vi "Analyze Code.vi"(11 "Test Case In":refnum<class "Runner Unit Test - Process Python Code.lvclass">) -> (0 "error out":errorcluster, 3 "Test Case Out":refnum<class "Runner Unit Test - Process Python Code.lvclass">)   [LabVIEW 2026, in "Runner Unit Test - Process Python Code.lvclass"]
uses:
  Runner Unit Test - Process Python Code.lvclass
  C:/Program Files/National Instruments/LabVIEW 2026/vi.lib/Astemes/LUnit/Test Case.lvclass
  Actors/Runner/Runner/Runner.lvclass
  Interfaces/IRunner/IRunner/Interfaces--cluster.ctl
  Interfaces/IProject Manager/IProject Manager.lvclass
  Interfaces/IFile Manager/IFile Manager.lvclass
  Interfaces/IPython Caller/IPython Caller.lvclass
  Interfaces/IElement Manager/IElement Manager.lvclass
  Interfaces/ILV File Creator/ILV File Creator.lvclass
  Interfaces/IHash Whitelist Handler/IHash Whitelist Handler.lvclass
  Actors/Mock Logger/Mock Logger/Mock Logger.lvclass
  C:/Program Files/National Instruments/LabVIEW 2026/vi.lib/ActorFramework/Actor/Actor.lvclass
  Type Definitions/Analysis Output--cluster.ctl
  Type Definitions/Type Definition--cluster.ctl
  Type Definitions/Parameter--cluster.ctl
  Type Definitions/Function--cluster.ctl
  <vilib>/ActorFramework/Message Enqueuer/Message Enqueuer.lvclass/Message Enqueuer.ctl
  <vilib>/ActorFramework/Message Enqueuer/Enqueue.vi
  Mocks/Mock IPython Caller/Mock IPython Caller.lvclass
  C:/Program Files/National Instruments/LabVIEW 2026/vi.lib/Astemes/LMock/Mock.lvclass
  C:/Users/juanj/Documents/hasbun_wood_engineering/github/py2vi/labview/Interfaces/IPython Caller/IPython Caller.lvclass
  <vilib>/ActorFramework/Stop Msg/Stop Msg.lvclass
  C:/Program Files/National Instruments/LabVIEW 2026/vi.lib/ActorFramework/Message/Message.lvclass
  <vilib>/Astemes/LMock/One Identical Inputs.vi
  <vilib>/ActorFramework/Message Priority Queue/Priority Enqueue.vi
  C:/Users/juanj/Documents/hasbun_wood_engineering/github/py2vi/labview/Mocks/Mock IPython Caller/Mock IPython Caller.lvclass
  Interfaces/IRunner/IRunner/IRunner.lvclass
  <vilib>/ActorFramework/Actor/Actor.lvclass
  <vilib>/Astemes/LMock/LMock Verifier.lvclass
  <vilib>/Astemes/LMock/LMock.lvlib
  <vilib>/Astemes/LMock/LMock One.lvlib
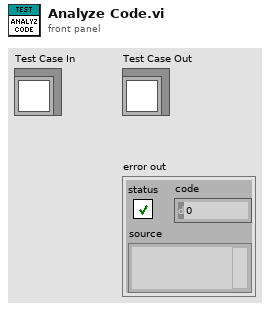
[diagram p1: front panel]
types:
  T1 = typedef "Function--cluster.ctl" = cluster{"name":string, "docstring":string, "input_parameters":T2[], "output_parameters":T2[]}
  T2 = typedef "Parameter--cluster.ctl" = cluster{"name":string, "data_type":string, "container":string, "dimensions":i32, "type_definition":string}
  T3 = typedef "Type Definition--cluster.ctl" = cluster{"name":string, "fields":T2[]}
  T4 = typedef "Analysis Output--cluster.ctl" = cluster{"type_definitions":T3[], "functions":T1[]}
  T5 = typedef "IRunner.lvlib/IRunner.lvclass/Interfaces--cluster.ctl" = cluster{"IProject Manager":refnum<class "IProject Manager.lvclass">, "IFile Manager":refnum<class "IFile Manager.lvclass">, "IPython Caller":refnum<class "IPython Caller.lvclass">, "IElement Manager":refnum<class "IElement Manager.lvclass">, "ILV File Creator":refnum<class "ILV File Creator.lvclass">, "IHash Whitelist Handler":refnum<class "IHash Whitelist Handler.lvclass">}
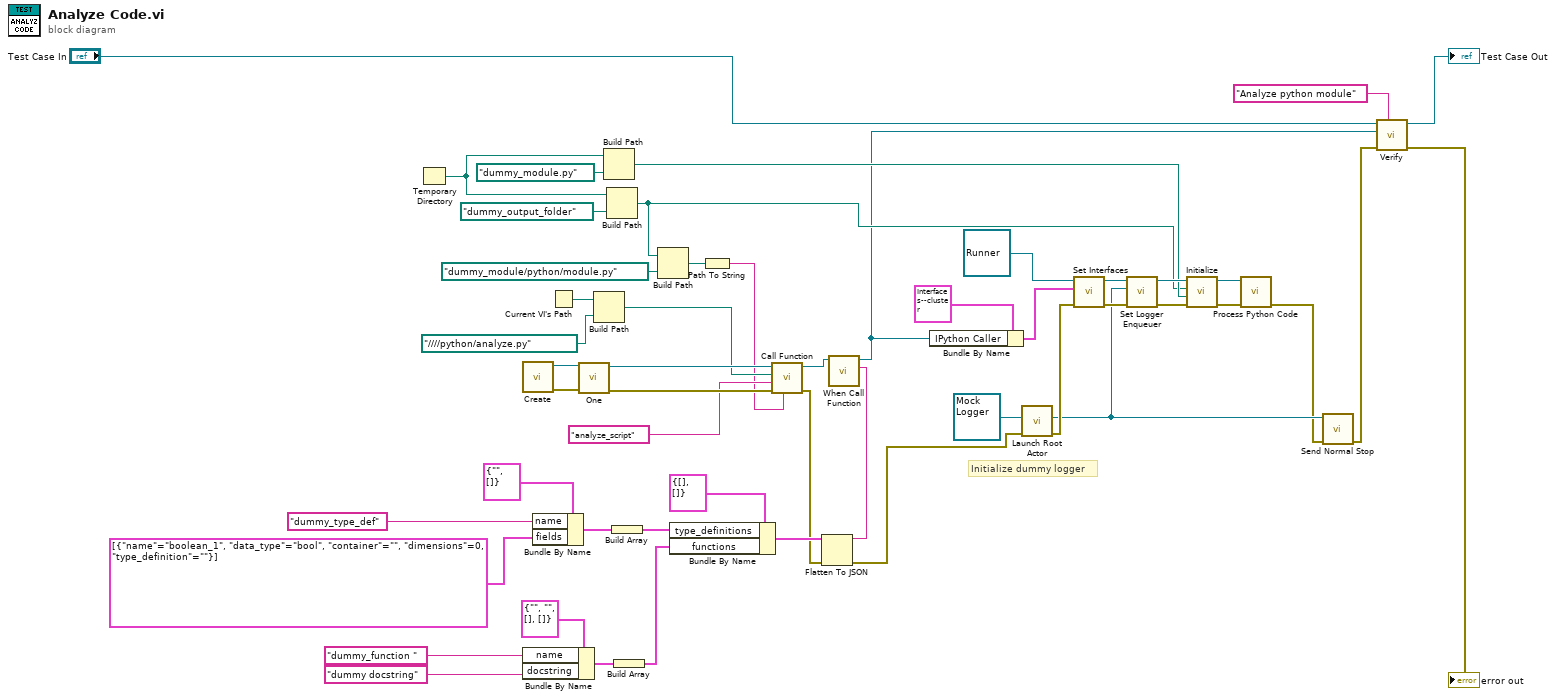
[diagram p0: block diagram]
diagram:
  # "Initialize dummy logger"
  n1 = Temporary Directory() -> (w36:path)
  n2 = call "Create.vi"() -> ("error out"=w30:errorcluster, "Mock Class Generator out"=w31:refnum<class "Mock IPython Caller.lvclass">)  [unwired: 10 in]
  n3 = Bundle By Name(cluster=T1 {"name"="", "docstring"="", "input_parameters"=[], "output_parameters"=[]} ("Function"), "name"="dummy_function ", "docstring"="dummy docstring") -> (w9:T1)
  n4 = Bundle By Name(cluster=T3 {"name"="", "fields"=[]} ("Type Definition"), "name"="dummy_type_def", "fields"=T2[] [{"name"="boolean_1", "data_type"="bool", "container"="", "dimensions"=0, "type_definition"=""}]) -> (w11:T3)
  n5 = Current VI's Path() -> (path=w26:path)
  n6 = call-poly <vilib>:"One.vi"("error in (no error)"=w30, "Mock in"=w31) -> ("error out"=w28:errorcluster, "Mock out"=w29:refnum<class "Mock IPython Caller.lvclass">)  [unwired: 8 in]
  n7 = Build Path(base path=w26, name or relative path=path "../../../../python/analyze.py") -> (appended path=w25:path)
  n8 = Build Path(base path=w36, name or relative path=path "dummy_module.py") -> (appended path=w37:path)
  n9 = Build Path(base path=w36, name or relative path=path "dummy_output_folder") -> (appended path=w23:path)
  n10 = Build Array(w11) -> (w10:T3[])
  n11 = Build Array(w9) -> (w8:T1[])
  n12 = Build Path(base path=w23, name or relative path=path "dummy_module/python/module.py") -> (appended path=w21:path)
  n13 = Bundle By Name(cluster=T4 {"type_definitions"=[], "functions"=[]} ("Analysis Output"), "type_definitions"=w10, "functions"=w8) -> (w7:T4)
  n14 = Path To String(path=w21) -> (string=w20:string)
  n15 = call-dynamic "Call Function.vi"("Input String"=w20, "error in"=w28, "Function"="analyze_script", "Python Script"=w25, "IPython Caller in"=w29) -> ("error out"=w4:errorcluster, "IPython Caller out"=w19:refnum<class "Mock IPython Caller.lvclass">)  [unwired: 4 in, 1 out]
  n16 = Flatten To JSON(anything=w7, error in (no error)=w4) -> (JSON string=w6:string, 11:w3:errorcluster)  [unwired: 1 in]
  n17 = call "When Call Function.vi"("Return String"=w6, "IPython Caller in"=w19) -> ("IPython Caller out"=w5:refnum<class "Mock IPython Caller.lvclass">)  [unwired: 9 in]
  n18 = Bundle By Name(cluster=T5 {"IProject Manager"=refnum, "IFile Manager"=refnum, "IPython Caller"=refnum, "IElement Manager"=refnum, "ILV File Creator"=refnum, "IHash Whitelist Handler"=refnum} ("Interfaces"), "IPython Caller"=w5) -> (w44:T5)
  n19 = call <vilib>:"Launch Root Actor.vi"("error in (no error)"=w3, "Actor"=refnum<class "Mock Logger.lvclass"> refnum ("Mock Logger.lvlib:Mock Logger.lvclass")) -> ("error out"=w50:errorcluster, "Actor's Enqueuer"=w42:refnum<class "Message Enqueuer.lvclass">)  [unwired: 8 in]
  n20 = call-dynamic "Set Interfaces.vi"("error in"=w50, "Interfaces"=w44, "Runner in"=refnum<class "Runner.lvclass"> refnum ("Runner.lvlib:Runner.lvclass")) -> ("error out"=w51:errorcluster, "Runner out"=w46:refnum<class "Runner.lvclass">)  [unwired: 7 in]
  n21 = call-dynamic "Set Logger Enqueuer.vi"("error in"=w51, "Logger"=w42, "Runner in"=w46) -> ("error out"=w48:errorcluster, "Runner out"=w39:refnum<class "Runner.lvclass">)  [unwired: 7 in]
  n22 = call-dynamic "Initialize.vi"("error in"=w48, "Python Module"=w37, "Output Folder"=w23, "G-CLI Runner in"=w39) -> ("error out"=w1:errorcluster, "G-CLI Runner out"=w2:refnum<class "Runner.lvclass">)  [unwired: 6 in]
  n23 = call-dynamic "Process Python Code.vi"("error in"=w1, "G-CLI Runner in"=w2) -> ("error out"=w32:errorcluster)  [unwired: 8 in, 1 out]
  n24 = call <vilib>:"Send Normal Stop.vi"("error in (no error)"=w32, "Message Enqueuer"=w42) -> ("error out"=w49:errorcluster)  [unwired: 9 in]
  n25 = call <vilib>:"Verify.vi"("Description"="Analyze python module", "error in (no error)"=w49, "Mock"=w5, "LUnit Test Case In"="Test Case In") -> ("error out"=→"error out":errorcluster, "LUnit Test Case Out"=→"Test Case Out":refnum<class "Runner Unit Test - Process Python Code.lvclass">)  [unwired: 6 in]
